vi "Confluence Settings Editor.vi"   [LabVIEW 2023]
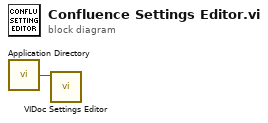
[diagram p0: block diagram]
diagram:
  n1 = call <vilib>:"Application Directory.vi"() -> ("Application Directory"=w1:path)
  n2 = call "VIDoc Settings Editor.vi"("VIDoc Settings Directory"=w1) -> ()  [unwired: 10 in, 1 out]
